vi "New Client.vi"(8 "error in (no error)":errorcluster, 9 "timeout ms (5000)":i32=5000, 11 "WebSocket URL":string) -> (0 "error out":errorcluster, 3 "WebSocket Client out":refnum<class "WebSocket Client.lvclass">)   [LabVIEW 2013, in "WebSockets.lvlib" / "WebSocket Client.lvclass"]
doc: "Opens a conenction and creates a new WebSocket Client using the NI VISA TCP Socket."
uses:
  WebSocket Client.lvclass
  WebSocket/WebSocket.lvclass/WebSocket.ctl
  WebSocket Client.lvclass/WebSocket Client.ctl
  WebSocket/Write Socket.vi
  Write URL.vi
  Sockets/VISA TCP Socket/VISA TCP.lvclass
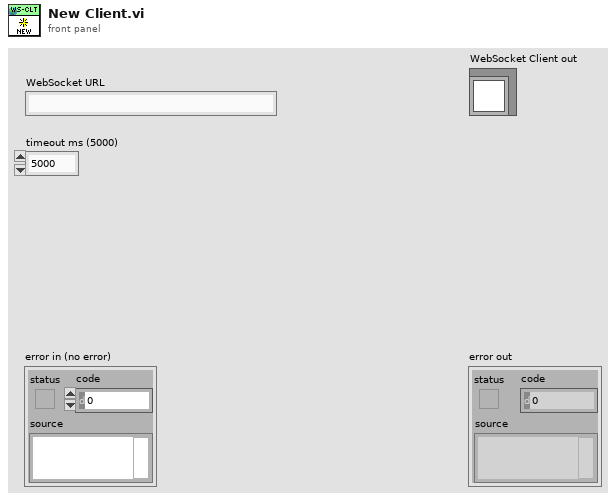
[diagram p1: front panel]
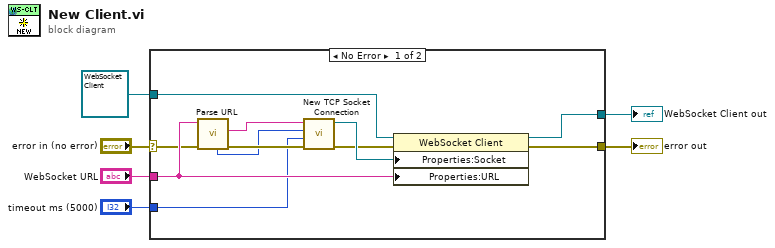
[diagram p0: block diagram]
diagram:
  n1 = case shown="No Error" "error in (no error)" {
    selector: "error in (no error)" -> [w13 w19]
    tunnel: refnum<class "WebSocket Client.lvclass"> refnum ("WebSocket Client in") -> [w17 w18]
    tunnel: [w16 w18] -> w5
    tunnel: [w15 w19] -> w4
    tunnel: "WebSocket URL" -> [w14 _]
    tunnel: "timeout ms (5000)" -> [w10 _]
    frame No Error {
      n2 = call "Parse URL.vi"("error in (no error)"=w13, "WebSocket URL"=w14) -> ("error out"=w12:errorcluster, "host"=w11:string, "port"=w9:u16)  [unwired: 5 in, 2 out]
      n3 = call "New TCP Socket Connection.vi"("error in (no error)"=w12, "timeout ms (5000)"=w10, "Port"=w9, "Hostname / IP"=w11) -> ("error out"=w7:errorcluster, "VISA TCP out"=w8:refnum<class "VISA TCP.lvclass">)  [unwired: 6 in]
      n4 = property class="WebSocket Client"(reference=w17, error in=w7, "Properties:Socket"=w8, "Properties:URL"=w14) -> (reference out=w16:refnum<class "WebSocket Client.lvclass">, error out=w15:errorcluster)
    }
    frame Error {
    }
  }
  "error out" <- w4
  "WebSocket Client out" <- w5
